vi "Initialize.vi"(7 "Project Store in":refnum<class "Project Store.lvclass">, 8 "error in (no error)":errorcluster, 11 "Data Folder":path) -> (0 "error out":errorcluster, 5 "Project Store out":refnum<class "Project Store.lvclass">)   [LabVIEW 2024, in "Project Store.lvclass"]
doc: "Prepares the store to use the given data folder. The parent class holds no storage location and does nothing here; a child class such as Project Store-INI overrides it and remembers the folder.\n\nGenerated by: Claude"
uses:
  Project Store.lvclass
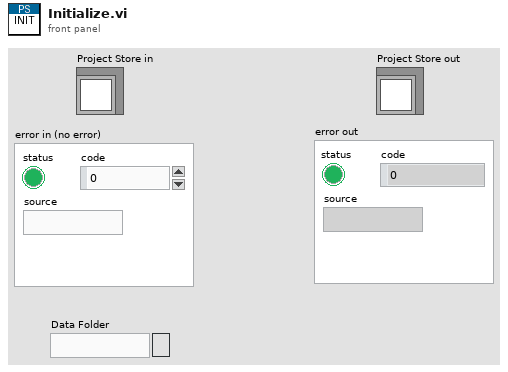
[diagram p1: front panel]
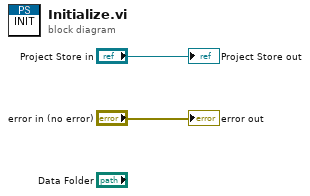
[diagram p0: block diagram]
diagram:
  "Project Store out" <- "Project Store in"
  "error out" <- "error in (no error)"
